vi "GpuMat Row.vi"(8 "error in (no error)":errorcluster, 10 "Y":i32, 11 "Src in":refnum<class "GpuMat.lvclass">) -> (0 "error out":errorcluster, 2 "Clone out":refnum<class "GpuMat.lvclass">, 3 "Src out":refnum<class "GpuMat.lvclass">)   [LabVIEW 2020, in "OpenLvVision_OpenCv.lvlib" / "Cuda.lvlib" / "GpuMat.lvclass"]
doc: "returns a new GpuMat header for the specified row"
uses:
  GpuMat.lvclass
  OpenLvVision_OpenCv.lvlib
  <vilib>/Utility/error.llb/Error Cluster From Error Code.vi
  <vilib>/ErrorRing/Error Ring.xnode
  _LvHelpers/EdvrObject/EdvrObject.lvclass
  _LvHelpers/EdvrObject/TypeDef/Edvr.ctl
  Dlls/OlvOpenCvWrapper.dll
  C:/Users/lukas/Documents/OpenLvVision_OpenCv/SourceCode/LabView/OpenLvVision_OpenCv/_LvHelpers/EdvrObject/EdvrObject.lvclass
  C:/Users/lukas/Documents/OpenLvVision_OpenCv/SourceCode/LabView/OpenLvVision_OpenCv/Cuda/DataAccess/GpuMat/GpuMat.lvclass
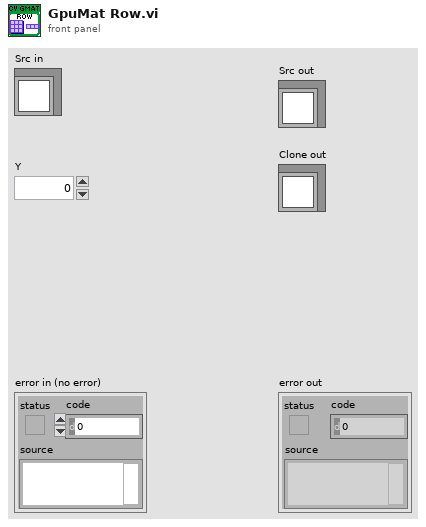
[diagram p1: front panel]
types:
  T1 = typedef "OpenLvVision_OpenCv.lvlib/EdvrObject.lvclass/Edvr.ctl" = refnum<data-value>
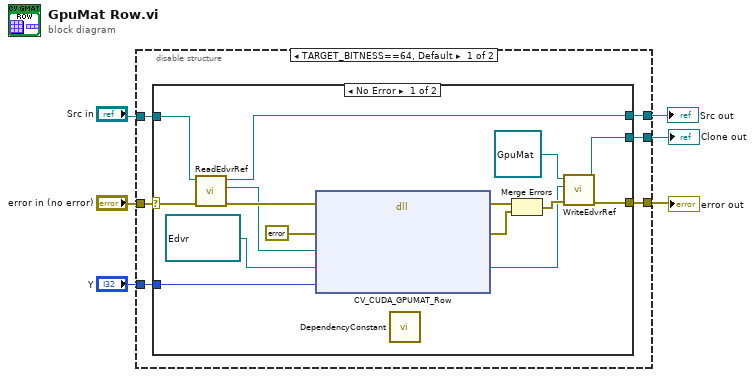
[diagram p0: block diagram]
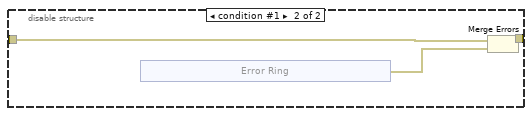
[diagram p3: hidden frame]
diagram:
  n1 = disable-structure shown="TARGET_BITNESS==64, Default" {
    disable-tunnel: "error in (no error)" -> [w12 w31]
    disable-tunnel: [w11 w32] -> w6
    disable-tunnel: "Src in" -> [w10 _]
    disable-tunnel: [w9 _] -> w3
    disable-tunnel: [w8 _] -> w2
    disable-tunnel: "Y" -> [w7 _]
    frame condition #0 (active) {
      n2 = case shown="No Error" w12 {
        selector: w12 -> [w20 w29]
        tunnel: [w18 w29] -> w11
        tunnel: w10 -> [w22 w28]
        tunnel: [w21 w28] -> w9
        tunnel: [w16 _] -> w8
        tunnel: w7 -> [w13 _]
        frame No Error {
          n3 = call "ReadEdvrRef.vi"("error in (no error)"=w20, "EdvrObject in"=w22) -> ("error out"=w24:errorcluster, "Edvr"=w23:T1, "EdvrObject out"=w21:refnum<class "GpuMat.lvclass">)  [unwired: 7 in]
          n4 = dll-call lib="C:/Users/lukas/Documents/OpenLvVision_OpenCv/SourceCode/LabView/OpenLvVision_OpenCv/Dlls/OlvOpenCvWrapper.dll" fn="CV_CUDA_GPUMAT_Row"(error in=w24, "Error"=errorcluster {"status"=FALSE, "code"=0, "source"=""} ("error out"), "srcRef"=w23, "dstRef"=T1 refnum ("Edvr"), "x"=w13) -> (error out=w27:errorcluster, "Error"=w26:errorcluster, "dstRef"=w15:T1)  [unwired: 5 in, 1 out]
          n5 = call "DependencyConstant.vi"() -> ()  [unwired: 12 in]
          n6 = Merge Errors(w27, w26) -> (w19:errorcluster)
          n7 = call "WriteEdvrRef.vi"("error in (no error)"=w19, "Edvr"=w15, "EdvrObject in"=refnum<class "GpuMat.lvclass"> refnum ("Dst out")) -> ("error out"=w18:errorcluster, "EdvrObject out"=w16:refnum<class "GpuMat.lvclass">)  [unwired: 7 in]
        }
        frame Error {
        }
      }
    }
    frame condition #1 {
      n8 = xnode "Error Ring"() -> ("error out"=w30:errorcluster)
      n9 = Merge Errors(w31, w30) -> (w32:errorcluster)
    }
  }
  "error out" <- w6
  "Clone out" <- w2
  "Src out" <- w3
